vi "CIVI Ensure LF.vi"(11 "Command":string) -> (3 "Terminated Command":string)   [LabVIEW 2026]
doc: "Returns Command unchanged if it already ends with LF.\nOtherwise, appends one LF byte (ASCII 10).\nDoes not interpret literal backslash-n text\nor normalize repeated trailing line endings."
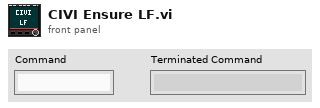
[diagram p1: front panel]
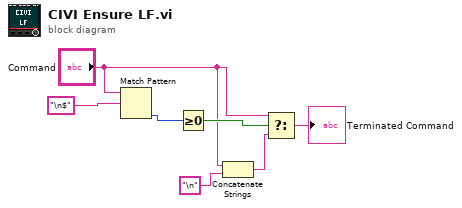
[diagram p0: block diagram]
diagram:
  n1 = Match Pattern(string="Command", regular expression="\n$") -> (offset past match=w6:i32)  [unwired: 1 in, 3 out]
  n2 = Greater Or Equal To 0?(x=w6) -> (x >= 0?=w5:bool)
  n3 = Concatenate Strings("Command", "\n" ("string")) -> (w3:string)
  n4 = Select(t="Command", s=w5, f=w3) -> (s? t:f=→"Terminated Command":string)
